vi "VIH ProjFile - Enum Info Array - Write.vi"(8 "error in":errorcluster, 9 "EnumValDscr":T1[](array[typedef]), 10 "Property Name":string, 11 "XML Parent Item":refnum<k20>) -> (0 "error out":errorcluster, 3 "dup XML Parent Item":refnum<k20>)   [LabVIEW 2014]
doc: "::: VI Helpeks :::\nCopyright (c) 2000-2026 Konstantin Shifershteyn. All rights reserved."
uses:
  _VIH HelpGen.llb/VIH HelpGen Typedef - Cluster - Enum Value Info.ctl
  <vilib>/xml/Close Reference(Node).vi
  <resource>/objmgr/DOMUserDefRef.rc
  <vilib>/xml/NI_XML.lvlib
panel:
  # "VI Helpeks\nCopyright (c) 2012-2026 Konstantin Shifershteyn"
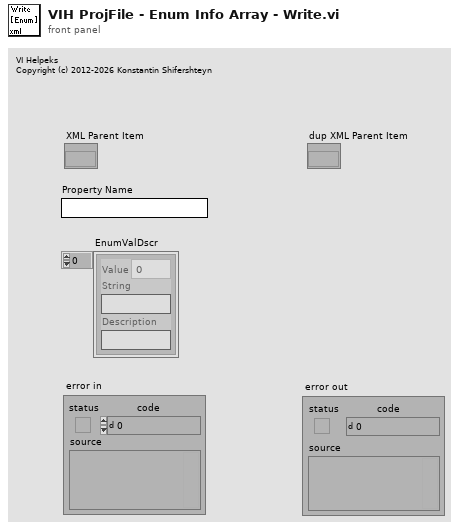
[diagram p1: front panel]
types:
  T1 = typedef "VIH HelpGen Typedef - Cluster - Enum Value Info.ctl" = cluster{"Value":ext, "String":string, "Description":string}
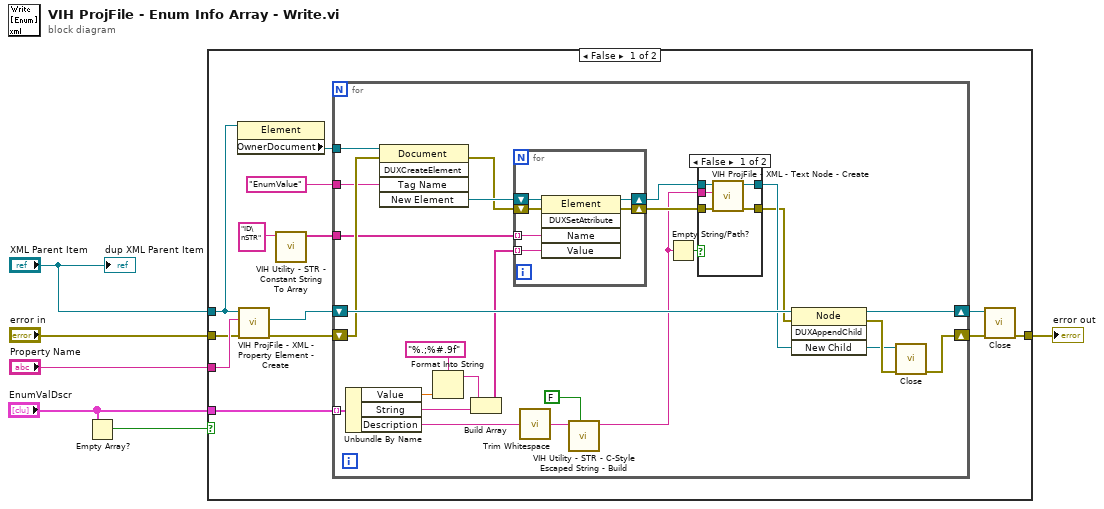
[diagram p0: block diagram]
diagram:
  n1 = Empty Array?(array="EnumValDscr") -> (empty?=w2:bool)
  n2 = case shown="False" w2 {
    tunnel: [w11 w58] -> w6
    tunnel: "XML Parent Item" -> [w10 _]
    tunnel: "Property Name" -> [w17 _]
    tunnel: "EnumValDscr" -> [w18 _]
    tunnel: "error in" -> [w13 w58]
    frame False {
      n3 = property class="Element"(reference=w10) -> ("OwnerDocument"=w14:refnum<k20>)  [unwired: 1 in, 2 out]
      n4 = call "VIH ProjFile - XML - Property Element - Create.vi"("error in"=w13, "Property Name"=w17, "XML Parent Item"=w10) -> ("error out"=w15:errorcluster, "New Child"=w16:refnum<k20>)  [unwired: 6 in, 1 out]
      n5 = call "VIH Utility - STR - Constant String To Array.vi"("String in"="ID\nSTR") -> ("Array out"=w7:string[])  [unwired: 10 in]
      n6 = for {
        shift-right: [w41] -> w12
        shift-left: w15 -> [w39]
        tunnel: w14 -> [w44]
        shift-right: [w42] -> w19
        shift-left: w16 -> [w43]
        tunnel: w18 -> [w38] mode=indexing
        tunnel: "EnumValue" ("Tag Name") -> [w37]
        tunnel: w7 -> [w34]
        n7 = Unbundle By Name(w38) -> ("Value"=w33:ext, "String"=w31:string, "Description"=w24:string)
        n8 = invoke class="Document" method="DUXCreateElement"(reference=w44, error in=w39, "Tag Name"=w37) -> (error out=w35:errorcluster, "New Element"=w36:refnum<k20>)  [unwired: 2 in, 3 out]
        n9 = Format Into String(format string="%.;%#.9f", w33) -> (resulting string=w30:string)  [unwired: 2 in, 1 out]
        n10 = Build Array(w30, w31) -> (w29:string[])
        n11 = for {
          tunnel: w29 -> [w52] mode=indexing
          shift-right: [w57] -> w28
          shift-left: w35 -> [w54]
          shift-right: [w56] -> w27
          shift-left: w36 -> [w55]
          tunnel: w34 -> [w53] mode=indexing
          n12 = invoke class="Element" method="DUXSetAttribute"(reference=w55, error in=w54, "Name"=w53, "Value"=w52) -> (reference out=w56:refnum<k20>, error out=w57:errorcluster)  [unwired: 1 in, 3 out]
        }
        n13 = call <vilib>:"Trim Whitespace.vi"("string"=w24) -> ("trimmed string"=w22:string)  [unwired: 1 in]
        n14 = call "VIH Utility - STR - C-Style Escaped String - Build.vi"("Escape space char (T)"=FALSE, "String in"=w22) -> ("String out"=w20:string)  [unwired: 9 in]
        n15 = Empty String/Path?(string/path=w20) -> (empty?=w23:bool)
        n16 = case shown="False" w23 {
          tunnel: w28 -> [w49 w50]
          tunnel: w27 -> [w48 w51]
          tunnel: [w47 w51] -> w26
          tunnel: [w46 w50] -> w25
          tunnel: w20 -> [w45 _]
          frame False {
            n17 = call "VIH ProjFile - XML - Text Node - Create.vi"("error in"=w49, "Data"=w45, "XML Parent Item"=w48) -> ("error out"=w46:errorcluster, "dup XML Parent Item"=w47:refnum<k20>)  [unwired: 7 in]
          }
          frame True {
          }
        }
        n18 = invoke class="Node" method="DUXAppendChild"(reference=w43, error in=w25, "New Child"=w26) -> (reference out=w42:refnum<k20>, error out=w40:errorcluster)  [unwired: 1 in, 2 out]
        n19 = call-poly <vilib>:"Close.vi"("error in (no error)"=w40, "node"=w26) -> ("error out"=w41:errorcluster)  [unwired: 7 in]
      }
      n20 = call-poly <vilib>:"Close.vi"("error in (no error)"=w12, "node"=w19) -> ("error out"=w11:errorcluster)  [unwired: 7 in]
    }
    frame True {
    }
  }
  "error out" <- w6
  "dup XML Parent Item" <- "XML Parent Item"
